vi "IDS Camera Engine.vi"(0 "IDS Notifier Name":string="Not a Name", 11 "Camera ID":string[](array[string])) -> ()   [LabVIEW 2016]
uses:
  IDS Controls/IDS Parameters.ctl
  IDS Controls/IDS Parameter List.ctl
  IDS Controls/IDS ROI.ctl
  IDS Controls/IDS Notifier Element.ctl
  IDS Controls/IDS Actions.ctl
  <vilib>/vision/Image Controls.llb/IMAQ Image.ctl
  C:/Users/user/Documents/Microscope-Control/Device Library/Cameras/IDS/IDS LabView Examples/LabVIEW/ueye.NET/uEyeDotNet.dll
  IDS LabView Examples/LabVIEW/ueye.NET/uEyeDotNet.dll
  Camera Controls/Camera IMAQ Key Info.ctl
panel:
  out "Image Key Error":errorcluster
  out "Frame":u32
  in  "Init Camera":bool
  in  "Quit":bool
  in  "Use Display Module":bool
  in  "Capture":bool
  in  "Live Preview":bool
  in  "Get ROI":bool
  in  "Set ROI":bool
  in  "Get Parameter":bool
  in  "Set Parameter":bool
  in  "File Save Path":path
  in  "# of Frames":u32
  in  "ROI Setup":T1
  in  "IDS Parameter":T2
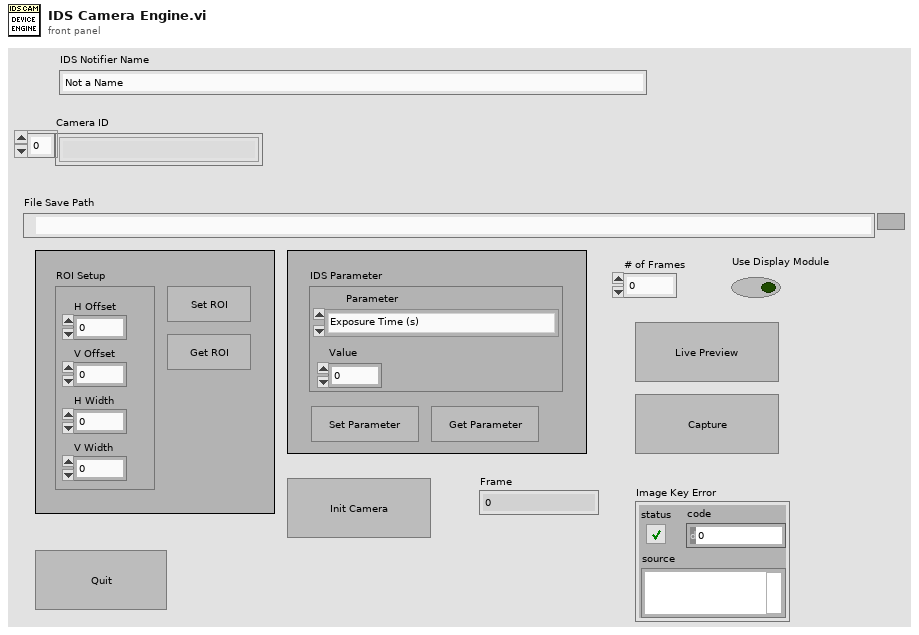
[diagram p1: front panel]
types:
  T1 = typedef "IDS ROI.ctl" = cluster{"H Offset":i32, "V Offset":i32, "H Width":i32, "V Width":i32}
  T2 = typedef "IDS Parameters.ctl" = cluster{"Parameter":T3, "Value":dbl}
  T3 = typedef "IDS Parameter List.ctl" = enum16{"Exposure Time (s)"}
  T4 = typedef "IDS Actions.ctl" = enum16{"Error Check", "Initialize", "Preview", "Record", "Abort", "Record Settings", "Set Parameter", "Get Parameter", "Set ROI", "Get ROI", "Status", "Quit"}
  T5 = typedef "Image Type" = u32
  T6 = typedef "IDS Notifier Element.ctl" = cluster{"IDS Actions":T4, "Received?":bool, "IDS Parameter":T2, "IDS ROI":T1, "Running?":bool, "File Path":path, "# of frames":u32, "Image Ref":T7, "Error":errorcluster}
  T7 = typedef "IMAQ Image.ctl" = refnum<image>
  T8 = typedef "Camera IMAQ Key Info.ctl" = cluster{"Frame":u32, "Sensor Height":i32, "Sensor Width":i32, "ROI Height":i32, "ROI Width":i32, "ROI Enable?":bool, "Bit per Pixel":u8}
  T9 = enum32{"Invalid", "Standard", "Closed", "Hidden", "Minimized", "Maximized"}
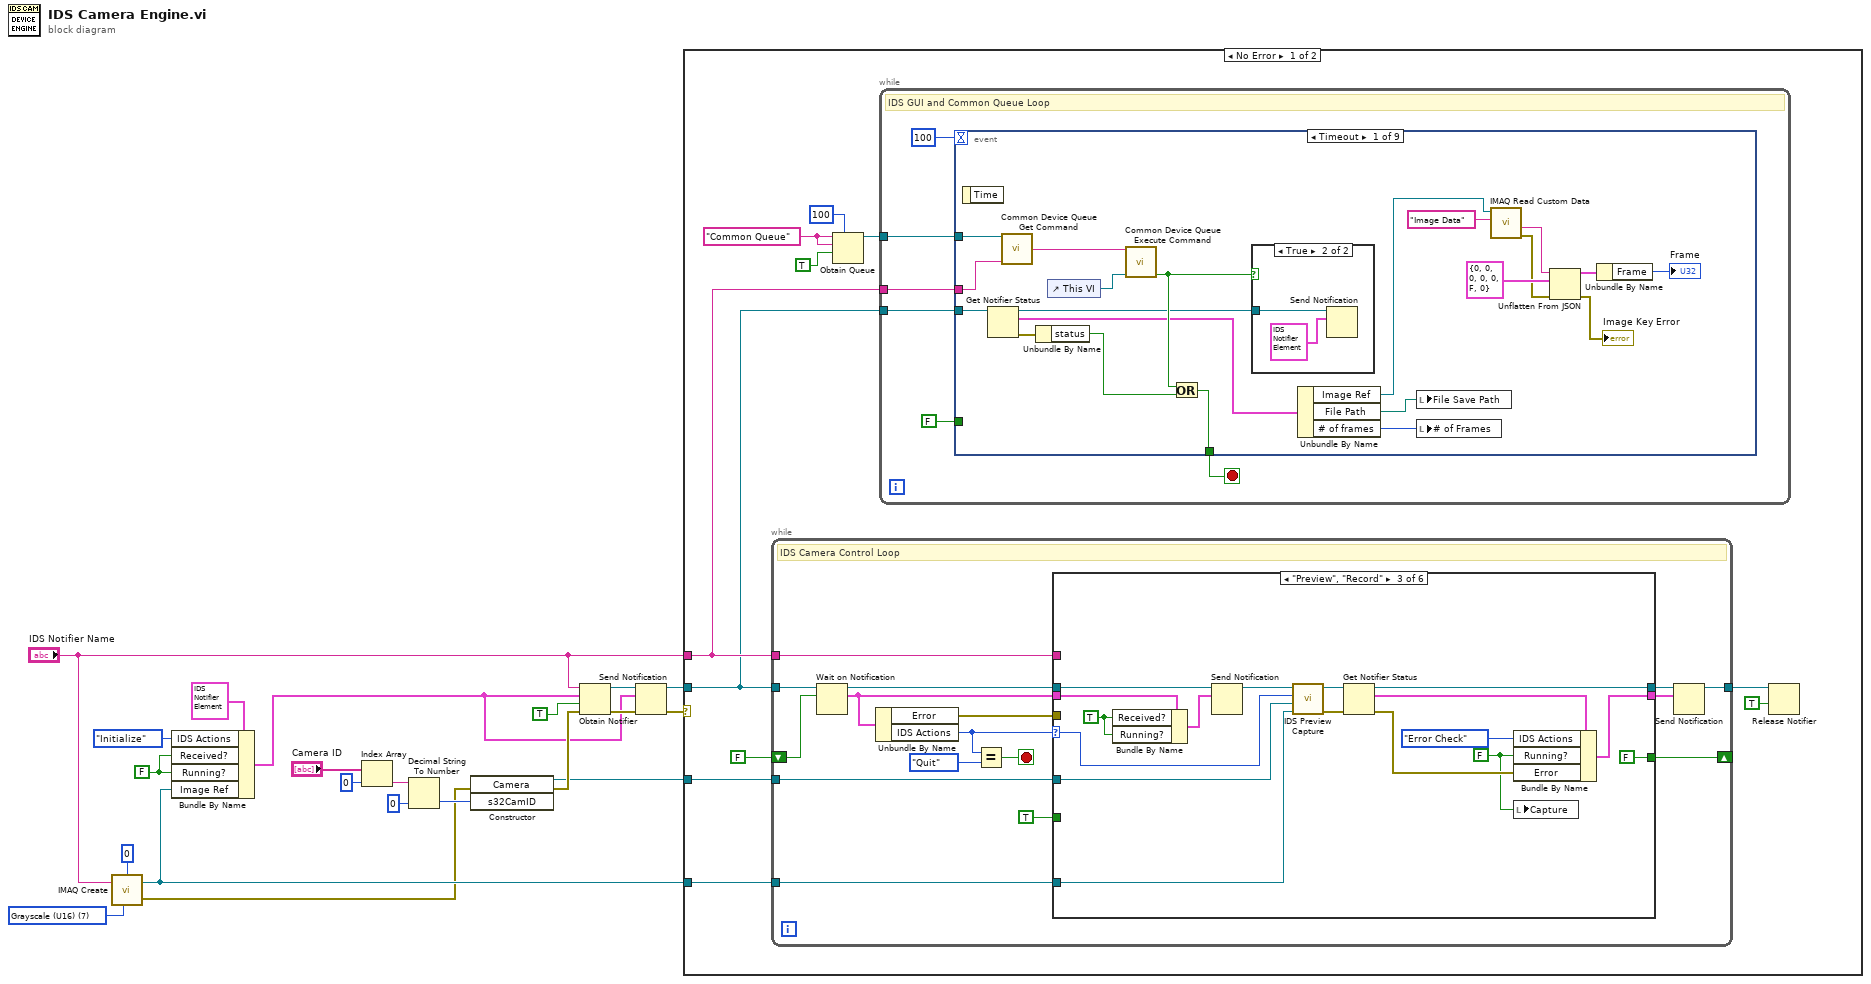
[diagram p0: block diagram]
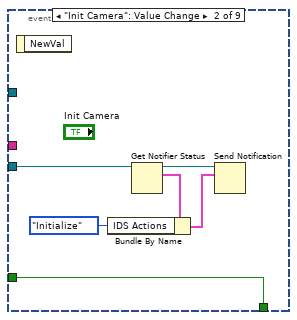
[diagram p3: hidden frame]
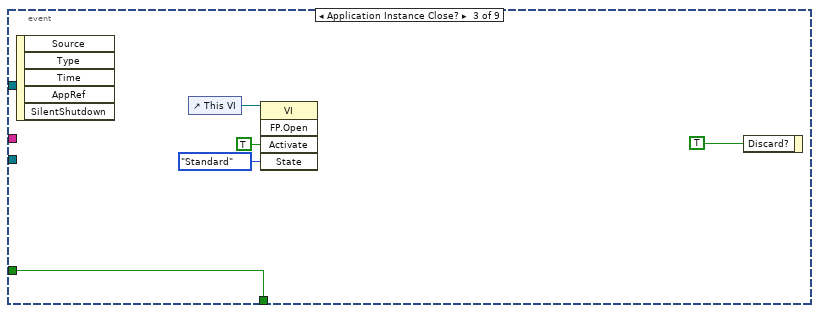
[diagram p4: hidden frame]
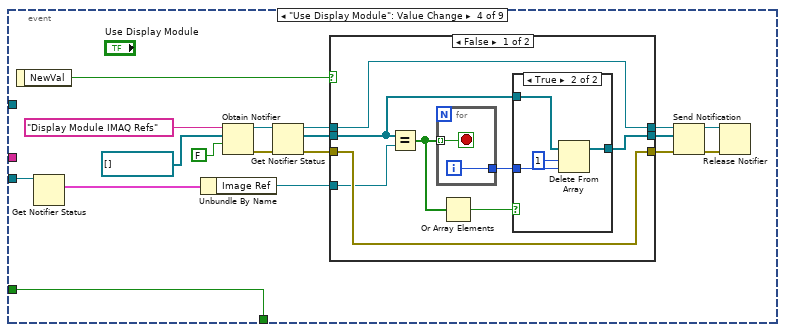
[diagram p5: hidden frame]
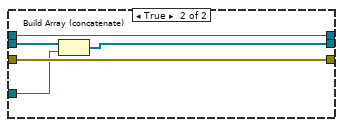
[diagram p7: hidden frame]
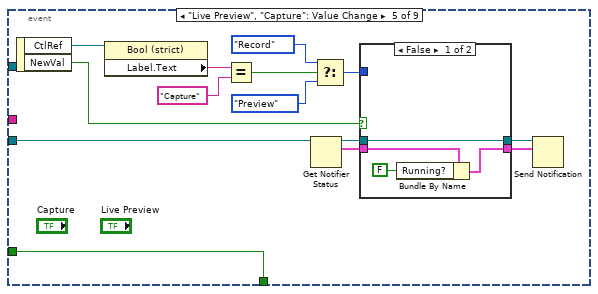
[diagram p8: hidden frame]
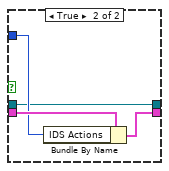
[diagram p9: hidden frame]
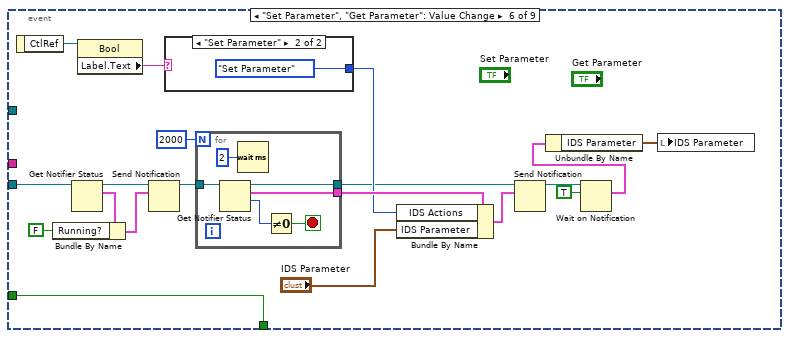
[diagram p10: hidden frame]
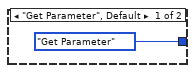
[diagram p11: hidden frame]
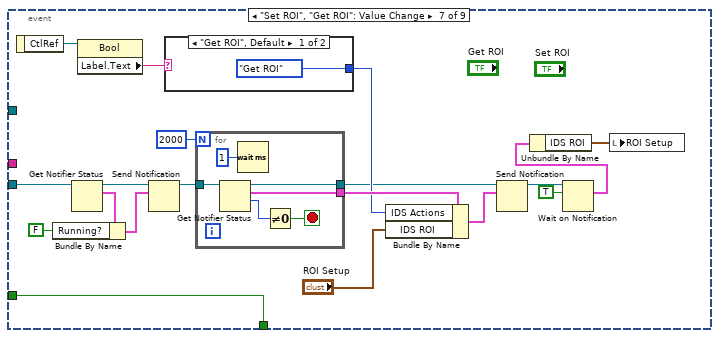
[diagram p12: hidden frame]
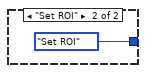
[diagram p13: hidden frame]
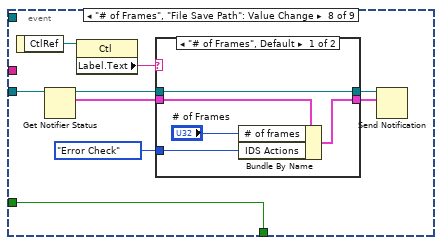
[diagram p14: hidden frame]
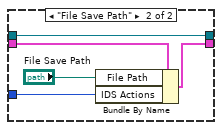
[diagram p15: hidden frame]
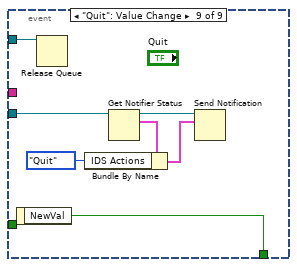
[diagram p16: hidden frame]
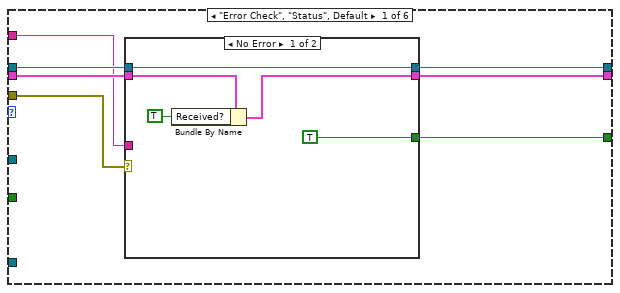
[diagram p17: hidden frame]
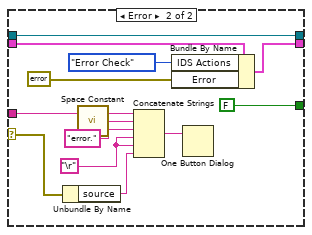
[diagram p18: hidden frame]
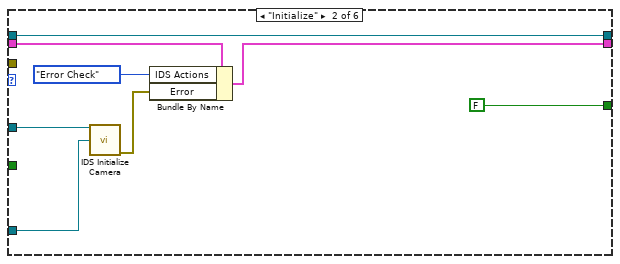
[diagram p19: hidden frame]
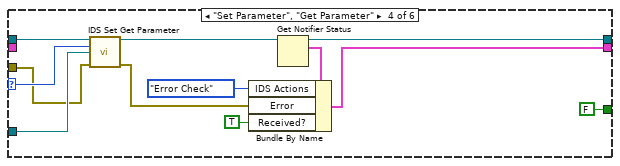
[diagram p20: hidden frame]
diagram:
  w5 = FALSE ("Received?")
  w10 = T5 7 items=["Grayscale (U8)", "Grayscale (I16)", "Grayscale (SGL)", "Complex (CSG)", "RGB (U32)", "HSL (U32)", "RGB (U64)", "Grayscale (U16)"] ("Image Type")
  n1 = call "IMAQ Create"("Border Size"=0, "Image Name"="IDS Notifier Name", "Image Type"=w10) -> ("New Image"=w2:T7, "error out"=w1:errorcluster)  [unwired: 2 in]
  n2 = Bundle By Name(cluster=T6 {"IDS Actions"=enum."Initialize", "Received?"=FALSE, "IDS Parameter"={"Parameter"=enum."Exposure Time (s)", "Value"=0.0}, "IDS ROI"={"H Offset"=0, "V Offset"=0, "H Width"=0, "V Width"=0}, "Running?"=FALSE, "File Path"=path "", "# of frames"=0, "Image Ref"=refnum, "Error"={"status"=FALSE, "code"=0, "source"=""}} ("IDS Camera Cluster"), "IDS Actions"=IDS_Actions."Initialize", "Received?"=w5, "Running?"=w5, "Image Ref"=w2) -> (w4:T6)
  n3 = Index Array(array="Camera ID", index=0) -> (element=w14:string)
  n4 = Decimal String To Number(string=w14, default (0L)=0 ("default (0 I32)")) -> (number=w12:i32)  [unwired: 1 in, 1 out]
  n5 = constructor class="Camera"(error in=w1, "s32CamID"=w12) -> (reference out=w3:refnum<k24>, error out=w9:errorcluster)  [unwired: 2 in, 2 out]
  n6 = Obtain Notifier(name (unnamed)="IDS Notifier Name", notification data type=w4, create if not found? (T)=TRUE, error in (no error)=w9) -> (notifier out=w20:refnum<notifier>, error out=w19:errorcluster)  [unwired: 1 out]
  n7 = Send Notification(notification=w4, notifier=w20, error in (no error)=w19) -> (notifier out=w18:refnum<notifier>, error out=w17:errorcluster)
  n8 = case shown="No Error" w17 {
    selector: w17 -> [_ w327]
    tunnel: w18 -> [w22 w328]
    tunnel: "IDS Notifier Name" -> [w23 w326]
    tunnel: w3 -> [w30 w319]
    tunnel: w2 -> [w29 w318]
    frame No Error {
      w27 = "Common Queue" ("Unique Notifier Name")
      n9 = while {
        tunnel: w22 -> [w226]
        tunnel: [w227] -> w31
        tunnel: w30 -> [w220]
        tunnel: w29 -> [w219]
        shift-right: [w216] -> _
        shift-left: FALSE -> [w218]
        tunnel: w23 -> [w214]
        stop <- w228 stop-if-true
        # "IDS Camera Control Loop"
        n10 = Wait on Notification(notifier=w226, ignore previous (F)=w218) -> (notifier out=w225:refnum<notifier>, notification=w224:T6)  [unwired: 2 in, 2 out]
        n11 = Unbundle By Name(w224) -> ("Error"=w213:errorcluster, "IDS Actions"=w223:T4)
        n12 = Equal?(x=w223, y=IDS_Actions."Quit") -> (x = y?=w228:bool)
        n13 = case shown="\"Preview\", \"Record\"" w223 {
          selector: w223 -> [_ _ w263 w284 w298 _]
          tunnel: w225 -> [w234 w261 w278 w280 w301 w313]
          tunnel: [w233 w261 w275 w289 w292 w313] -> w221
          tunnel: w224 -> [w232 w259 w277 _ _ w311]
          tunnel: w214 -> [w231 _ _ _ _ _]
          tunnel: w220 -> [_ w260 w264 w283 w300 w307]
          tunnel: w219 -> [_ w254 w265 _ w299 w305]
          tunnel: [w230 w256 w274 w285 w291 w309] -> w217
          tunnel: [w235 FALSE FALSE FALSE w302 w312] -> w216
          tunnel: TRUE -> [_ _ _ _ w302 w312]
          tunnel: w213 -> [w229 _ _ w282 _ w303]
          frame "Error Check", "Status", Default {
            n14 = case shown="No Error" w229 {
              selector: w229 -> [_ w243]
              tunnel: w232 -> [w238 w253]
              tunnel: [TRUE FALSE] -> w235
              tunnel: [w240 w250] -> w233
              tunnel: w234 -> [w240 w250]
              tunnel: w231 -> [_ w249]
              tunnel: [w236 w245] -> w230
              frame No Error {
                n15 = Bundle By Name(cluster=w238, "Received?"=TRUE) -> (w236:T6)
              }
              frame Error {
                w244 = "\r"
                n16 = Unbundle By Name(w243) -> ("source"=w242:string)
                n17 = call <vilib>:"Space Constant.vi"() -> ("String"=w248:string)
                n18 = Concatenate Strings(w249, w248, "error." ("string"), w244, w244, w242) -> (w246:string)
                n19 = Bundle By Name(cluster=w253, "IDS Actions"=IDS_Actions."Error Check", "Error"=errorcluster {"status"=FALSE, "code"=0, "source"=""}) -> (w245:T6)
                n20 = One Button Dialog(message=w246) -> ()  [unwired: 1 in, 1 out]
              }
            }
          }
          frame "Initialize" {
            n21 = call "IDS Initialize Camera.vi"("Camera ID"=w260, "IDS Cam Img Ref"=w254) -> ("Error Out"=w257:errorcluster)  [unwired: 12 in, 1 out]
            n22 = Bundle By Name(cluster=w259, "IDS Actions"=IDS_Actions."Error Check", "Error"=w257) -> (w256:T6)
          }
          frame "Preview", "Record" {
            w262 = FALSE ("Running?")
            w271 = TRUE ("Received?")
            n23 = Bundle By Name(cluster=w277, "Received?"=w271, "Running?"=w271) -> (w273:T6)
            n24 = Send Notification(notification=w273, notifier=w278) -> (notifier out=w270:refnum<notifier>)  [unwired: 1 in, 1 out]
            n25 = call "IDS Preview Capture.vi"("Image Ref"=w265, "IDS Camera Ref"=w264, "IDS Actions"=w263, "IDS Notifier"=w270) -> ("Error"=w267:errorcluster, "IDS Notifier"=w269:refnum<notifier>)  [unwired: 6 in]
            n26 = Get Notifier Status(notifier=w269, error in (no error)=w267) -> (notifier out=w275:refnum<notifier>, current notification=w268:T6, error out=w266:errorcluster)  [unwired: 2 out]
            n27 = Bundle By Name(cluster=w268, "IDS Actions"=IDS_Actions."Error Check", "Running?"=w262, "Error"=w266) -> (w274:T6)
            n28 = local write "Capture"(w262) -> ()
          }
          frame "Set Parameter", "Get Parameter" {
            n29 = call "IDS Set Get Parameter.vi"("IDS Notifier"=w280, "IDS Actions"=w284, "IDS Camera Ref"=w283, "Error"=w282) -> ("IDS Notifier"=w290:refnum<notifier>, "Error"=w286:errorcluster)  [unwired: 10 in]
            n30 = Get Notifier Status(notifier=w290) -> (notifier out=w289:refnum<notifier>, current notification=w288:T6)  [unwired: 1 in, 3 out]
            n31 = Bundle By Name(cluster=w288, "IDS Actions"=IDS_Actions."Error Check", "Error"=w286, "Received?"=TRUE) -> (w285:T6)
          }
          frame "Set ROI", "Get ROI" {
            n32 = call "IDS Set Get ROI.vi"("IDS Notifier Ref"=w301, "IDS Actions"=w298, "IDS Camera Ref"=w300, "IDS Image Ref"=w299) -> ("IDS Notifier Ref (Dup)"=w293:refnum<notifier>, "Error"=w294:errorcluster)  [unwired: 10 in]
            n33 = Get Notifier Status(notifier=w293) -> (notifier out=w292:refnum<notifier>, current notification=w297:T6)  [unwired: 1 in, 3 out]
            n34 = Bundle By Name(cluster=w297, "IDS Actions"=IDS_Actions."Error Check", "Error"=w294, "Received?"=TRUE) -> (w291:T6)
          }
          frame "Quit" {
            n35 = call "IMAQ Dispose"("Image"=w305) -> ()  [unwired: 5 in, 1 out]
            n36 = invoke class="Camera" method="Exit"(reference=w307, error in=w303) -> (reference out=w308:refnum<k24>, error out=w306:errorcluster)  [unwired: 1 in, 1 out]
            n37 = Close Reference(reference=w308, error in (no error)=w306) -> (error out=w304:errorcluster)
            n38 = Bundle By Name(cluster=w311, "Received?"=TRUE, "Error"=w304) -> (w309:T6)
          }
        }
        n39 = Send Notification(notification=w217, notifier=w221) -> (notifier out=w227:refnum<notifier>)  [unwired: 1 in, 1 out]
      }
      n40 = Obtain Queue(max queue size (-1, unlimited)=100, name (unnamed)=w27, element data type=w27, create if not found? (T)=TRUE) -> (queue out=w24:refnum<queue>)  [unwired: 1 in, 2 out]
      n41 = while {
        tunnel: w24 -> [w37]
        tunnel: w23 -> [w35]
        tunnel: w22 -> [w36]
        stop <- w34 stop-if-true
        # "IDS GUI and Common Queue Loop"
        n42 = event shown="[0] Timeout" {
          selector: _ -> [_ _ _ _ _ _ _ _ _]
          dyn-events: _ -> [_ _ _ _ _ _ _ _ _]
          timeout: 100 -> [_ _ _ _ _ _ _ _ _]
          tunnel: w37 -> [w53 _ _ _ _ _ _ _ w212]
          tunnel: w36 -> [w52 w66 _ w90 w115 w149 w176 w193 w211]
          tunnel: w35 -> [w51 _ _ _ _ _ _ _ _]
          tunnel: [w50 w67 w72 w73 w124 w151 w178 w195 w206] -> w34
          tunnel: FALSE -> [_ w67 w72 w73 w124 w151 w178 w195 _]
          event Timeout {
            n43 = event-data() -> ()  [unwired: 1 in, 1 out]
            n44 = Get Notifier Status(notifier=w52) -> (notifier out=w54:refnum<notifier>, current notification=w47:T6, error out=w59:errorcluster)  [unwired: 1 in, 2 out]
            n45 = call "Common Device Queue Get Command.vi"("Common Queue"=w53, "Notifier Name"=w51) -> ("Command"=w58:string)  [unwired: 12 in, 1 out]
            n46 = Unbundle By Name(w59) -> ("status"=w56:bool)
            n47 = control-ref of="This VI"() -> (w57:refnum<vi>)
            n48 = call "Common Device Queue Execute Command.vi"("Common Command"=w58, "VI Refnum"=w57) -> ("Quit?"=w55:bool)  [unwired: 12 in, 1 out]
            n49 = Or(x=w55, y=w56) -> (x .or. y?=w50:bool)
            n50 = case shown="True" w55 {
              tunnel: w54 -> [_ w61]
              frame False {
              }
              frame True {
                n51 = Send Notification(notification=T6 {"IDS Actions"=enum."Quit", "Received?"=FALSE, "IDS Parameter"={"Parameter"=enum."Exposure Time (s)", "Value"=0.0}, "IDS ROI"={"H Offset"=0, "V Offset"=0, "H Width"=0, "V Width"=0}, "Running?"=FALSE, "File Path"=path "", "# of frames"=0, "Image Ref"=refnum, "Error"={"status"=FALSE, "code"=0, "source"=""}} ("IDS Camera Cluster"), notifier=w61) -> ()  [unwired: 1 in, 2 out]
              }
            }
            n52 = Unbundle By Name(w47) -> ("Image Ref"=w45:T7, "File Path"=w49:path, "# of frames"=w48:u32)
            n53 = local write "File Save Path"(w49) -> ()
            n54 = local write "# of Frames"(w48) -> ()
            n55 = call "IMAQ Read Custom Data"("Key"="Image Data", "Image"=w45) -> ("error out"=w40:errorcluster, "Custom Data Out"=w43:string)  [unwired: 7 in, 1 out]
            n56 = Unflatten From JSON(JSON string=w43, type and defaults=T8 {"Frame"=0, "Sensor Height"=0, "Sensor Width"=0, "ROI Height"=0, "ROI Width"=0, "ROI Enable?"=FALSE, "Bit per Pixel"=0} ("Camera IMAQ Key Info"), error in (no error)=w40) -> (value=w42:T8, error out=→"Image Key Error":errorcluster)  [unwired: 4 in]
            n57 = Unbundle By Name(w42) -> ("Frame"=→"Frame":u32)
          }
          event "Init Camera": Value Change {
            n58 = event-data() -> ()  [unwired: 1 in, 1 out]
            n59 = Get Notifier Status(notifier=w66) -> (notifier out=w62:refnum<notifier>, current notification=w65:T6)  [unwired: 1 in, 3 out]
            n60 = Bundle By Name(cluster=w65, "IDS Actions"=IDS_Actions."Initialize") -> (w63:T6)
            n61 = Send Notification(notification=w63, notifier=w62) -> ()  [unwired: 1 in, 2 out]
          }
          event Application Instance Close? {
            n62 = event-data() -> ()  [unwired: 1 in, 5 out]
            n63 = control-ref of="This VI"() -> (w69:refnum<vi>)
            n64 = invoke class="VI" method="FP.Open"(reference=w69, "Activate"=TRUE ("Activate?"), "State"=T9."Standard") -> ()  [unwired: 2 in, 5 out]
            n65 = event-data("Discard?"=TRUE) -> ()  [unwired: 1 in, 1 out]
          }
          event "Use Display Module": Value Change {
            n66 = event-data() -> ("NewVal"=w75:bool)  [unwired: 1 in]
            n67 = Get Notifier Status(notifier=w90) -> (current notification=w89:T6)  [unwired: 1 in, 4 out]
            n68 = Unbundle By Name(w89) -> ("Image Ref"=w74:T7)
            n69 = Obtain Notifier(name (unnamed)="Display Module IMAQ Refs", notification data type=T7[] [], create if not found? (T)=FALSE) -> (notifier out=w82:refnum<notifier>, error out=w81:errorcluster)  [unwired: 1 in, 1 out]
            n70 = Get Notifier Status(notifier=w82, error in (no error)=w81) -> (notifier out=w83:refnum<notifier>, current notification=w85:T7[], error out=w84:errorcluster)  [unwired: 2 out]
            n71 = case shown="False" w75 {
              tunnel: w83 -> [w98 w108]
              tunnel: w84 -> [w92 w107]
              tunnel: w85 -> [w94 w110]
              tunnel: [w93 w109] -> w88
              tunnel: [w98 w108] -> w86
              tunnel: [w92 w107] -> w87
              tunnel: w74 -> [w91 w106]
              frame False {
                n72 = Equal?(x=w94, y=w91) -> (x = y?=w97:bool[])
                n73 = for {
                  tunnel: w97 -> [w105] mode=indexing
                  tunnel: [w104] -> w95
                  i -> [w104]
                  stop <- w105 stop-if-true
                }
                n74 = Or Array Elements(Boolean array=w97) -> (logical OR=w96:bool)
                n75 = case shown="True" w96 {
                  tunnel: w95 -> [_ w102]
                  tunnel: w94 -> [w99 w101]
                  tunnel: [w99 w100] -> w93
                  frame False {
                  }
                  frame True {
                    n76 = Delete From Array(array=w101, length=1, index=w102) -> (array with subset deleted=w100:T7[])  [unwired: 1 out]
                  }
                }
              }
              frame True {
                n77 = Build Array (concatenate)(w110, w106) -> (w109:T7[])
              }
            }
            n78 = Send Notification(notification=w88, notifier=w86, error in (no error)=w87) -> (notifier out=w80:refnum<notifier>, error out=w79:errorcluster)
            n79 = Release Notifier(notifier=w80, error in (no error)=w79) -> ()  [unwired: 1 in, 3 out]
          }
          event "Live Preview", "Capture": Value Change {
            n80 = event-data() -> ("CtlRef"=w123:refnum<vi>, "NewVal"=w117:bool)  [unwired: 1 in]
            n81 = property class="Bool (strict)"(reference=w123) -> ("Label.Text"=w122:string)  [unwired: 1 in, 2 out]
            n82 = Equal?(x=w122, y="Capture") -> (x = y?=w120:bool)
            n83 = Get Notifier Status(notifier=w115) -> (notifier out=w114:refnum<notifier>, current notification=w113:T6)  [unwired: 1 in, 3 out]
            n84 = Select(t=IDS_Actions."Record" ("y"), s=w120, f=IDS_Actions."Preview" ("y")) -> (s? t:f=w116:T4)
            n85 = case shown="False" w117 {
              tunnel: w116 -> [_ w131]
              tunnel: w114 -> [w126 w130]
              tunnel: w113 -> [w128 w132]
              tunnel: [w126 w130] -> w112
              tunnel: [w125 w129] -> w111
              frame False {
                n86 = Bundle By Name(cluster=w128, "Running?"=FALSE) -> (w125:T6)
              }
              frame True {
                n87 = Bundle By Name(cluster=w132, "IDS Actions"=w131) -> (w129:T6)
              }
            }
            n88 = Send Notification(notification=w111, notifier=w112) -> ()  [unwired: 1 in, 2 out]
          }
          event "Set Parameter", "Get Parameter": Value Change {
            n89 = event-data() -> ("CtlRef"=w150:refnum<vi>)  [unwired: 1 in]
            n90 = Get Notifier Status(notifier=w149) -> (notifier out=w144:refnum<notifier>, current notification=w147:T6)  [unwired: 1 in, 3 out]
            n91 = Bundle By Name(cluster=w147, "Running?"=FALSE) -> (w143:T6)
            n92 = property class="Bool"(reference=w150) -> ("Label.Text"=w148:string)  [unwired: 1 in, 2 out]
            n93 = Send Notification(notification=w143, notifier=w144) -> (notifier out=w142:refnum<notifier>)  [unwired: 1 in, 1 out]
            n94 = case shown="\"Set Parameter\"" w148 {
              tunnel: [IDS_Actions."Get Parameter" ("IDS Actions") IDS_Actions."Set Parameter" ("IDS Actions")] -> w139
              frame "Get Parameter", Default {
              }
              frame "Set Parameter" {
              }
            }
            n95 = for {
              N: 2000 -> [_]
              tunnel: w142 -> [w156]
              tunnel: [w155] -> w138
              tunnel: [w154] -> w141
              stop <- w152 stop-if-true
              n96 = Get Notifier Status(notifier=w156) -> (notifier out=w155:refnum<notifier>, current notification=w154:T6, # waiting=w153:i32)  [unwired: 1 in, 2 out]
              n97 = Wait (ms)(milliseconds to wait=u32 2) -> ()  [unwired: 1 out]
              n98 = Not Equal To 0?(x=w153) -> (x != 0?=w152:bool)
            }
            n99 = Bundle By Name(cluster=w141, "IDS Actions"=w139, "IDS Parameter"="IDS Parameter") -> (w137:T6)
            n100 = Send Notification(notification=w137, notifier=w138) -> (notifier out=w136:refnum<notifier>)  [unwired: 1 in, 1 out]
            n101 = Wait on Notification(notifier=w136, ignore previous (F)=TRUE) -> (notification=w134:T6)  [unwired: 2 in, 3 out]
            n102 = Unbundle By Name(w134) -> ("IDS Parameter"=w133:T2)
            n103 = local write "IDS Parameter"(w133) -> ()
          }
          event "Set ROI", "Get ROI": Value Change {
            n104 = event-data() -> ("CtlRef"=w177:refnum<vi>)  [unwired: 1 in]
            n105 = Get Notifier Status(notifier=w176) -> (notifier out=w171:refnum<notifier>, current notification=w174:T6)  [unwired: 1 in, 3 out]
            n106 = Bundle By Name(cluster=w174, "Running?"=FALSE) -> (w170:T6)
            n107 = property class="Bool"(reference=w177) -> ("Label.Text"=w175:string)  [unwired: 1 in, 2 out]
            n108 = Send Notification(notification=w170, notifier=w171) -> (notifier out=w169:refnum<notifier>)  [unwired: 1 in, 1 out]
            n109 = case shown="\"Get ROI\", Default" w175 {
              tunnel: [IDS_Actions."Get ROI" ("IDS Actions") IDS_Actions."Set ROI" ("IDS Actions")] -> w167
              frame "Get ROI", Default {
              }
              frame "Set ROI" {
              }
            }
            n110 = for {
              N: 2000 -> [_]
              tunnel: w169 -> [w183]
              tunnel: [w182] -> w166
              tunnel: [w181] -> w168
              stop <- w179 stop-if-true
              n111 = Get Notifier Status(notifier=w183) -> (notifier out=w182:refnum<notifier>, current notification=w181:T6, # waiting=w180:i32)  [unwired: 1 in, 2 out]
              n112 = Wait (ms)(milliseconds to wait=u32 1) -> ()  [unwired: 1 out]
              n113 = Not Equal To 0?(x=w180) -> (x != 0?=w179:bool)
            }
            n114 = Bundle By Name(cluster=w168, "IDS Actions"=w167, "IDS ROI"="ROI Setup") -> (w165:T6)
            n115 = Send Notification(notification=w165, notifier=w166) -> (notifier out=w164:refnum<notifier>)  [unwired: 1 in, 1 out]
            n116 = Wait on Notification(notifier=w164, ignore previous (F)=TRUE) -> (notification=w162:T6)  [unwired: 2 in, 3 out]
            n117 = Unbundle By Name(w162) -> ("IDS ROI"=w161:T1)
            n118 = local write "ROI Setup"(w161) -> ()
          }
          event "# of Frames", "File Save Path": Value Change {
            n119 = event-data() -> ("CtlRef"=w194:refnum<vi>)  [unwired: 1 in]
            n120 = Get Notifier Status(notifier=w193) -> (notifier out=w191:refnum<notifier>, current notification=w190:T6)  [unwired: 1 in, 3 out]
            n121 = property class="Ctl"(reference=w194) -> ("Label.Text"=w192:string)  [unwired: 1 in, 2 out]
            n122 = case shown="\"# of Frames\", Default" w192 {
              tunnel: w191 -> [w198 w205]
              tunnel: w190 -> [w200 w204]
              tunnel: [w198 w205] -> w189
              tunnel: [w197 w203] -> w188
              tunnel: IDS_Actions."Error Check" ("IDS Actions") -> [w196 w201]
              frame "# of Frames", Default {
                n123 = Bundle By Name(cluster=w200, "# of frames"="# of Frames", "IDS Actions"=w196) -> (w197:T6)
              }
              frame "File Save Path" {
                n124 = Bundle By Name(cluster=w204, "File Path"="File Save Path", "IDS Actions"=w201) -> (w203:T6)
              }
            }
            n125 = Send Notification(notification=w188, notifier=w189) -> ()  [unwired: 1 in, 2 out]
          }
          event "Quit": Value Change {
            n126 = event-data() -> ("NewVal"=w206:bool)  [unwired: 1 in]
            n127 = Release Queue(queue=w212) -> ()  [unwired: 2 in, 3 out]
            n128 = Get Notifier Status(notifier=w211) -> (notifier out=w210:refnum<notifier>, current notification=w209:T6)  [unwired: 1 in, 3 out]
            n129 = Bundle By Name(cluster=w209, "IDS Actions"=IDS_Actions."Quit") -> (w207:T6)
            n130 = Send Notification(notification=w207, notifier=w210) -> ()  [unwired: 1 in, 2 out]
          }
        }
      }
      n131 = Release Notifier(notifier=w31, force destroy? (F)=TRUE) -> ()  [unwired: 1 in, 3 out]
    }
    frame Error {
      n132 = Release Notifier(notifier=w328, force destroy? (F)=TRUE, error in (no error)=w327) -> (error out=w317:errorcluster)  [unwired: 2 out]
      n133 = invoke class="Camera" method="Exit"(reference=w319, error in=w317) -> (reference out=w320:refnum<k24>, error out=w316:errorcluster)  [unwired: 1 in, 1 out]
      n134 = Close Reference(reference=w320, error in (no error)=w316) -> (error out=w315:errorcluster)
      n135 = call "IMAQ Dispose"("Image"=w318, "error in (no error)"=w315) -> ("error out"=w314:errorcluster)  [unwired: 4 in]
      n136 = Unbundle By Name(w314) -> ("source"=w321:string)
      n137 = call <vilib>:"Space Constant.vi"() -> ("String"=w324:string)
      n138 = Concatenate Strings(w326, w324, "Device Error." ("string"), "\r", w321) -> (w325:string)
      n139 = One Button Dialog(message=w325) -> ()  [unwired: 1 in, 1 out]
    }
  }
